vi "channel qualification test.vi"() -> (0 "no err":errorcluster, 3 "qualified channels OK":bool)   [LabVIEW 2014, in "TEC tests.lvlib"]
uses:
  TEC tests.lvlib
  <vilib>/NI/Configuration Framework/serializable configuration/NISE_CEF_serializable configuration.lvclass/NISE_CEF_serializable configuration.ctl
  <vilib>/NI/Tag Bus/tag/tag descriptor.lvclass/tag descriptor.ctl
  <vilib>/NI/Configuration Framework/serializable configuration/Read UID.vi
  <vilib>/Utility/LVClass/Get LV Class Name.vi
  <vilib>/NI/Configuration Framework/error generator/NISE_error generator.vi
  <vilib>/NI/Tag Bus/tag/tag descriptor.lvclass
  <vilib>/NI/Tag Bus Module Framework/channel/TBM channel.lvclass
  <vilib>/NI/Tag Bus Module Framework/module configuration/TBM module configuration.lvclass
  configuration/TEC configuration.lvclass
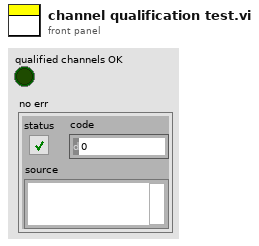
[diagram p1: front panel]
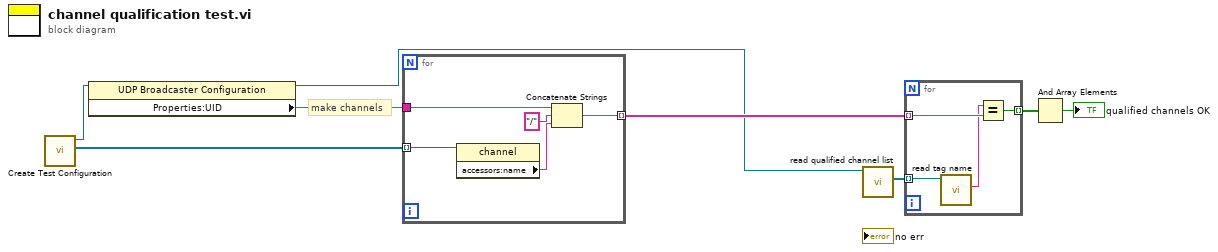
[diagram p0: block diagram]
diagram:
  # "make channels"
  n1 = call "Create Test Configuration.vi"() -> ("Array"=w2:refnum<class "TBM channel.lvclass">[], "TEC configuration out"=w4:refnum<class "TEC configuration.lvclass">)  [unwired: 8 in, 2 out]
  n2 = property class="UDP Broadcaster Configuration"(reference=w4) -> (reference out=w1:refnum<class "TEC configuration.lvclass">, "Properties:UID"=w3:string)  [unwired: 1 in, 1 out]
  n3 = for {
    tunnel: w2 -> [w13] mode=indexing
    tunnel: w3 -> [w12]
    tunnel: [w11] -> w5 mode=indexing
    n4 = property class="channel"(reference=w13) -> ("accessors:name"=w9:string)  [unwired: 1 in, 2 out]
    n5 = Concatenate Strings(w12, "/" ("string"), w9) -> (w11:string)
  }
  n6 = call <vilib>:"read qualified channel list.vi"("module configuration in"=w1) -> ("qualified channels"=w6:refnum<class "TBM channel.lvclass">[])  [unwired: 9 in, 1 out]
  n7 = for {
    tunnel: w5 -> [w16] mode=indexing
    tunnel: w6 -> [w17] mode=indexing
    tunnel: [w14] -> w8 mode=indexing
    n8 = call <vilib>:"read tag name.vi"("system tag in"=w17) -> ("name"=w15:string)  [unwired: 8 in, 2 out]
    n9 = Equal?(x=w15, y=w16) -> (x = y?=w14:bool)
  }
  n10 = And Array Elements(Boolean array=w8) -> (logical AND=→"qualified channels OK":bool)
